vi "RDV-addDataToGraph-name.vi"(8 "error in (no error)":errorcluster, 11 "RDV-Reflection_Data_viewer in":refnum<class "RDV-Reflection_Data_viewer.lvclass">) -> (0 "error out":errorcluster, 3 "RDV-Reflection_Data_viewer out":refnum<class "RDV-Reflection_Data_viewer.lvclass">)   [LabVIEW 2020, in "RDV-Reflection_Data_viewer.lvclass"]
doc: "Writes the plot names of the viewer's data to the graphs."
uses:
  RDV-Reflection_Data_viewer.lvclass
  RDV-Reflection_Data_viewer.lvclass/RDV-Reflection_Data_viewer.ctl
  <vilib>/regexp/Match Regular Expression.xnode
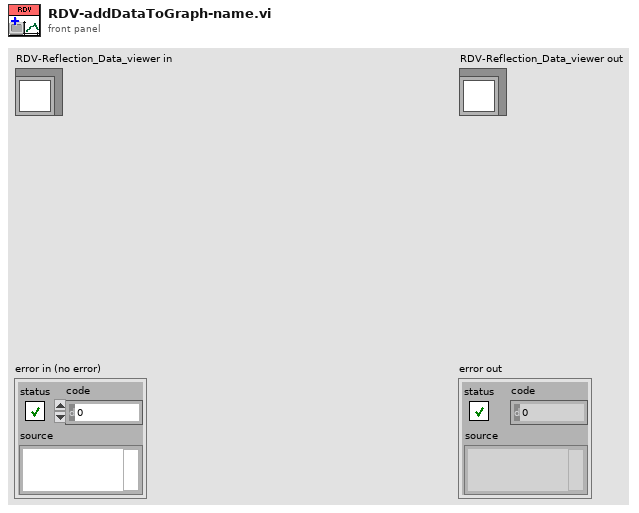
[diagram p1: front panel]
types:
  T1 = typedef "RDV-Reflection_Data_viewer.lvclass/RDV-XY_GRAPH_REFS.ctl" = cluster{"Reflection Real":refnum<vi>, "Reflection Imag":refnum<vi>, "Permittivity Real":refnum<vi>, "Permittivity Imag":refnum<vi>, "Impedance Real":refnum<vi>, "Impedance Imag":refnum<vi>}
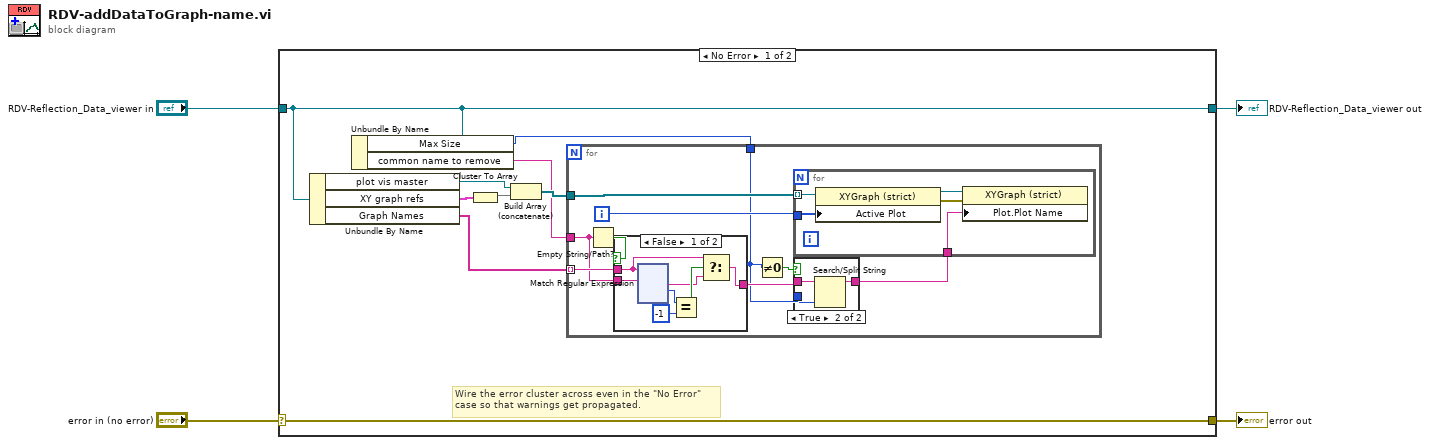
[diagram p0: block diagram]
diagram:
  n1 = case shown="No Error" "error in (no error)" {
    selector: "error in (no error)" -> [w13 w155]
    tunnel: [w13 w155] -> w3
    tunnel: [w7 w154] -> w1
    tunnel: "RDV-Reflection_Data_viewer in" -> [w7 w154]
    frame No Error {
      # "Wire the error cluster across even in the \"No Error\"\ncase so that warnings get propagated."
      n2 = Unbundle By Name(w7) -> ("plot vis master"=w8:refnum<vi>, "XY graph refs"=w10:T1, "Graph Names"=w12:string[])
      n3 = Unbundle By Name(w7) -> ("Max Size"=w6:i32, "common name to remove"=w5:string)
      n4 = Cluster To Array(cluster=w10) -> (array=w11:refnum<vi>[])
      n5 = Build Array (concatenate)(w8, w11) -> (w9:refnum<vi>[])
      n6 = for {
        tunnel: w9 -> [w21]
        tunnel: w12 -> [w16] mode=indexing
        tunnel: w6 -> [w17]
        tunnel: w5 -> [w14]
        i -> [w22]
        n7 = Empty String/Path?(string/path=w14) -> (empty?=w15:bool)
        n8 = case shown="False" w15 {
          tunnel: w16 -> [w24 w144]
          tunnel: w14 -> [w29 _]
          tunnel: [w23 w144] -> w20
          frame False {
            n9 = xnode "Match Regular Expression"("input string"=w24, "regular expression"=w29) -> ("after match"=w25:string, "offset past match"=w28:i32)  [unwired: 4 in, 3 out]
            n10 = Equal?(x=w28, y=-1) -> (x = y?=w26:bool)
            n11 = Select(t=w24, s=w26, f=w25) -> (s? t:f=w23:string)
          }
          frame True {
          }
        }
        n12 = Not Equal To 0?(x=w17) -> (x != 0?=w18:bool)
        n13 = case shown="True" w18 {
          tunnel: w17 -> [_ w148]
          tunnel: w20 -> [w145 w147]
          tunnel: [w145 w146] -> w19
          frame False {
          }
          frame True {
            n14 = Search/Split String(string=w147, offset (0)=w148) -> (substring before match=w146:string)  [unwired: 1 in, 2 out]
          }
        }
        n15 = for {
          tunnel: w22 -> [w153]
          tunnel: w19 -> [w152]
          tunnel: w21 -> [w151] mode=indexing
          n16 = property on="Property Node" class="XYGraph (strict)"(reference=w151, "Active Plot"=w153) -> (reference out=w150:refnum<vi>, error out=w149:errorcluster)  [unwired: 1 in]
          n17 = property on="Property Node" class="XYGraph (strict)"(reference=w150, error in=w149, "Plot.Plot Name"=w152) -> ()  [unwired: 2 out]
        }
      }
    }
    frame Error {
    }
  }
  "error out" <- w3
  "RDV-Reflection_Data_viewer out" <- w1
